vi "Get Test Registration by Key.vi"(8 "error in (no error)":errorcluster, 10 "Key":string, 11 "Test Event Storage in":refnum<class "Test Event Storage.lvclass">) -> (0 "error out":errorcluster, 1 "Test Node":T1={"Test Registration"={"Name"="", "Call Chain"=[], "Time Stamp"=timestamp(0 s since 1904-01-01), "Test ID"="", "Caller ID"=""}, "Defined"=TRUE, "Passed"=TRUE}, 2 "Found?":bool, 3 "Test Event Storage out":refnum<class "Test Event Storage.lvclass">)   [LabVIEW 2013, in "Caraya.lvlib" / "Test Event Storage.lvclass"]
uses:
  Test Event Storage.lvclass
  Test Result/Test Node.ctl
  Test Result/Test Registration Data.ctl
  Test Event Storage.lvclass/Test Event Storage.ctl
  test store -- cluster.ctl
  Test Manager Message Test/TestManagerMsg.Test.lvclass
  Test Result/Test Result.lvclass
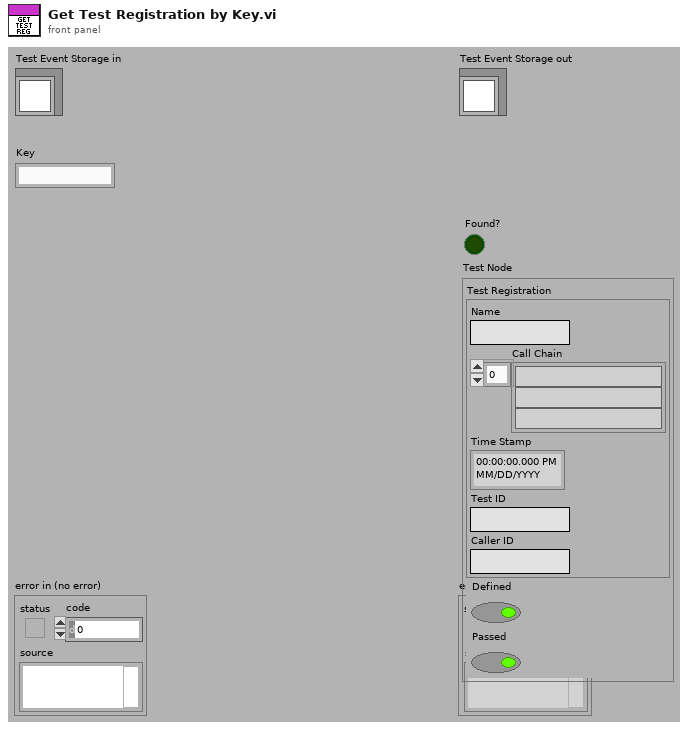
[diagram p1: front panel]
types:
  T1 = typedef "Caraya.lvlib/Test Result.lvclass/Test Node.ctl" = cluster{"Test Registration":T2, "Defined":bool, "Passed":bool}
  T2 = typedef "Caraya.lvlib/Test Result.lvclass/Test Registration Data.ctl" = cluster{"Name":string, "Call Chain":string[], "Time Stamp":timestamp, "Test ID":string, "Caller ID":string}
  T3 = typedef "Caraya.lvlib/Test Event Storage.lvclass/test store -- cluster.ctl" = cluster{"Test":refnum<class "TestManagerMsg.Test.lvclass">, "Defined":bool, "Passed":bool, "properties":variant, "assert-ids":variant}
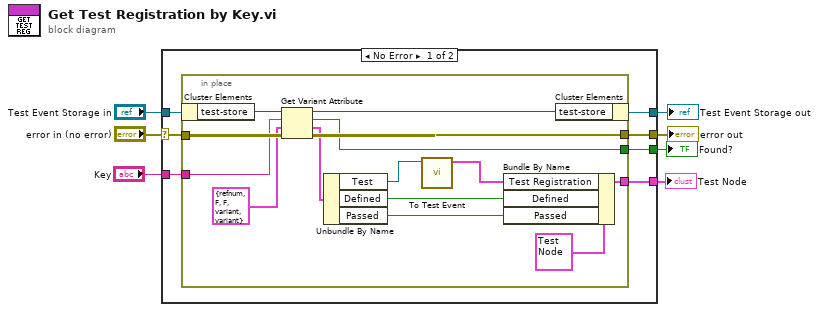
[diagram p0: block diagram]
diagram:
  n1 = case shown="No Error" "error in (no error)" {
    selector: "error in (no error)" -> [w10 w30]
    tunnel: [w14 w30] -> w6
    tunnel: [w13 w29] -> w4
    tunnel: "Test Event Storage in" -> [w8 w29]
    tunnel: [w12 _] -> w1
    tunnel: "Key" -> [w11 _]
    tunnel: [w9 _] -> w2
    frame No Error {
      n2 = in-place {
        in-place-border: w10 -> [w27]
        in-place-border: [w24] -> w14
        in-place-border: [w17] -> w12
        in-place-border: w11 -> [w23]
        in-place-border: [w22] -> w9
        n3 = in-place-cluster #1(w8) -> ("test-store"=w28:variant)
        n4 = Get Variant Attribute(Variant=w28, name=w23, default value (empty Variant)=T3 {"Test"=refnum, "Defined"=FALSE, "Passed"=FALSE, "properties"=variant, "assert-ids"=variant} ("test-store"), error in=w27) -> (duplicate Variant=w26:variant, found=w22:bool, value=w25:T3, error out=w24:errorcluster)
        n5 = Unbundle By Name(w25) -> ("Test"=w20:refnum<class "TestManagerMsg.Test.lvclass">, "Defined"=w16:bool, "Passed"=w15:bool)
        n6 = call "To Test Event.vi"("TestManagerMsg.Test in"=w20) -> ("Test Registration"=w18:T2)  [unwired: 10 in]
        n7 = Bundle By Name(cluster=T1 {"Test Registration"={"Name"="", "Call Chain"=[], "Time Stamp"=timestamp(0 s since 1904-01-01), "Test ID"="", "Caller ID"=""}, "Defined"=TRUE, "Passed"=TRUE} ("Test Node"), "Test Registration"=w18, "Defined"=w16, "Passed"=w15) -> (w17:T1)
        n8 = in-place-cluster #1("test-store"=w26) -> (w13:refnum<class "Test Event Storage.lvclass">)
      }
    }
    frame Error {
    }
  }
  "error out" <- w6
  "Test Event Storage out" <- w4
  "Test Node" <- w1
  "Found?" <- w2
